vi "Destroy_MemBank.vi"(8 "error in":errorcluster, 11 "NNPC_MemBank_and_Params":T1={"MemBank_Data"={"MemBank"=variant, "MemBank Norm"=variant}, "PreProc_Options"={"DS_Name"="", "Input_Dims"={"C"=-1, "H"=-1, "W"=-1}, "Cropping"={"Left"=0.0, "Top"=0.0, "Right"=1.0, "Bottom"=1.0}, "Interpolation Type"=1, "MultiStage_ReSample?"=FALSE, "Dataset_Stats"={"means"={"R"=0.5385, "G"=0.5348, "B"=0.551}, "stds"={"R"=0.3673, "G"=0.3673, "B"=0.3505}}}, "Evaluation_Results"={"Threshold(Image)"=0.0, "Threshold(Pixel)"=0.0, "Pixel_Range"={"Min"=0.0, "Max"=0.0}}, "MemBank on GPU?"=FALSE} {"PreProc_Options"."Dataset_Stats"."stds"."R" format="%#_3g"; "PreProc_Options"."Dataset_Stats"."stds"."G" format="%#_3g"; "PreProc_Options"."Dataset_Stats"."stds"."B" format="%#_3g"; "PreProc_Options"."Dataset_Stats"."means"."R" format="%#_3g"; "PreProc_Options"."Dataset_Stats"."means"."G" format="%#_3g"; "PreProc_Options"."Dataset_Stats"."means"."B" format="%#_3g"; "PreProc_Options"."Interpolation Type" items=["Zero Order", "Bi-Linear", "Quadratic", "Cubic Spline"]; "Evaluation_Results"."Pixel_Range"."Min" format="%#_5g"}) -> (0 "error out":errorcluster)   [LabVIEW 2020]
uses:
  <vilib>/Ngene/DeepLTK Anomaly Detection Addon/Toolkit/API/Controls/MemBank_and_Norm_Variants.ctl
  <vilib>/Ngene/CuLab - GPU Accelerated Toolkit/Toolkit/Low_Level/Tensor_Classes/T_Children/T1D/T1D_Children/T1D_SGL/T1D_SGL.lvclass
  C:/Program Files/National Instruments/LabVIEW 2020/vi.lib/Ngene/CuLab - GPU Accelerated Toolkit/Toolkit/Low_Level/Tensor_Classes/Tensor.lvclass
  <vilib>/Ngene/CuLab - GPU Accelerated Toolkit/Toolkit/Low_Level/Tensor_Classes/T_Children/T2D/T2D_Children/T2D_SGL/T2D_SGL.lvclass
  <vilib>/Ngene/Deep Learning Toolkit/Toolkit/Deep_Learning_Toolkit_by_Ngene.lvlib
  <vilib>/Ngene/CuLab - GPU Accelerated Toolkit/Toolkit/CuLab.lvlib
  <vilib>/Ngene/DeepLTK Anomaly Detection Addon/Toolkit/DeepLTK_Anomaly_Detection_Addon.lvlib
  <vilib>/Ngene/DeepLTK Anomaly Detection Addon/Toolkit/API/Controls/NNPC_Evaluation_Results.ctl
  <vilib>/Ngene/Deep Learning Toolkit/Toolkit/NN_Data/API/NN_Dims(C,H,W).ctl
  <vilib>/Ngene/DeepLTK Anomaly Detection Addon/Toolkit/API/Controls/Image_Stats_RGB.ctl
  <vilib>/Ngene/DeepLTK Anomaly Detection Addon/Toolkit/API/Controls/NNPC_DS_Stats.ctl
  <vilib>/Ngene/DeepLTK Anomaly Detection Addon/Toolkit/API/Controls/Crop_CFG.ctl
  <vilib>/Ngene/DeepLTK Anomaly Detection Addon/Toolkit/API/Controls/NNPC_PreProcessing_Options.ctl
  Controls/NNPC_MemBank_and_Params.ctl
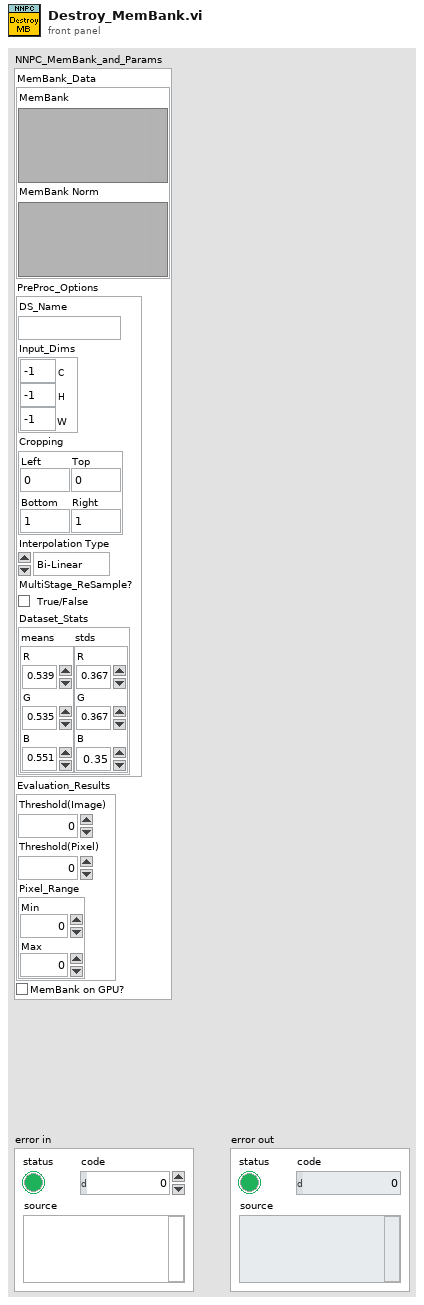
[diagram p1: front panel]
types:
  T1 = typedef "NNPC_MemBank_and_Params.ctl" = cluster{"MemBank_Data":T2, "PreProc_Options":T3, "Evaluation_Results":T8, "MemBank on GPU?":bool}
  T2 = typedef "DeepLTK_Anomaly_Detection_Addon.lvlib/MemBank_and_Norm_Variants.ctl" = cluster{"MemBank":variant, "MemBank Norm":variant}
  T3 = typedef "DeepLTK_Anomaly_Detection_Addon.lvlib/NNPC_PreProcessing_Options.ctl" = cluster{"DS_Name":string, "Input_Dims":T4, "Cropping":T5, "Interpolation Type":u32, "MultiStage_ReSample?":bool, "Dataset_Stats":T6}
  T4 = typedef "Deep_Learning_Toolkit_by_Ngene.lvlib/NN_Dims(C,H,W).ctl" = cluster{"C":i32, "H":i32, "W":i32}
  T5 = typedef "DeepLTK_Anomaly_Detection_Addon.lvlib/Crop_CFG.ctl" = cluster{"Left":sgl, "Top":sgl, "Right":sgl, "Bottom":sgl}
  T6 = typedef "DeepLTK_Anomaly_Detection_Addon.lvlib/NNPC_DS_Stats.ctl" = cluster{"means":T7, "stds":T7}
  T7 = typedef "DeepLTK_Anomaly_Detection_Addon.lvlib/Image_Stats_RGB.ctl" = cluster{"R":sgl, "G":sgl, "B":sgl}
  T8 = typedef "DeepLTK_Anomaly_Detection_Addon.lvlib/NNPC_Evaluation_Results.ctl" = cluster{"Threshold(Image)":sgl, "Threshold(Pixel)":sgl, "Pixel_Range":cluster{"Min":sgl, "Max":sgl}}
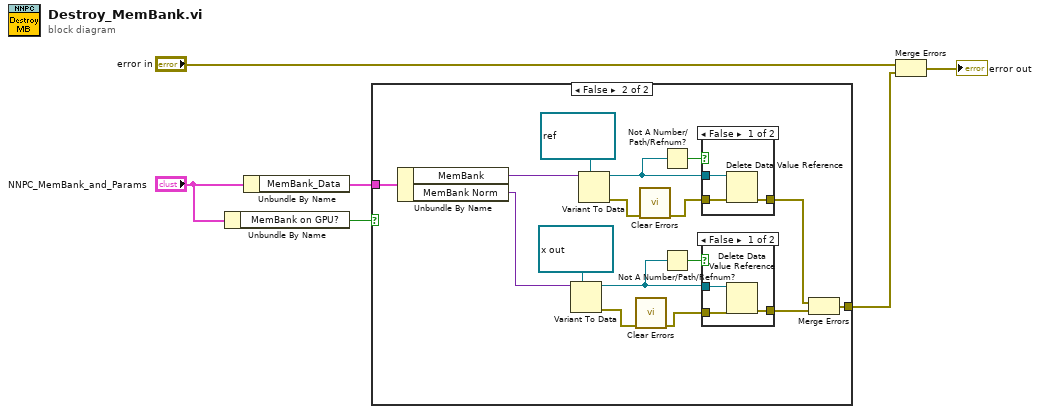
[diagram p0: block diagram]
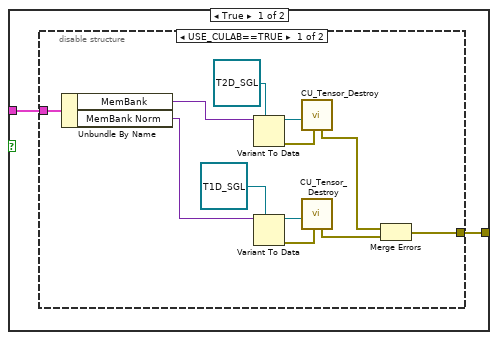
[diagram p2: hidden frame]
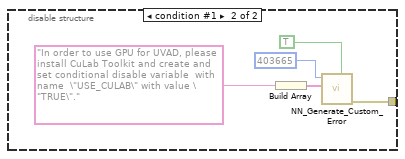
[diagram p3: hidden frame]
diagram:
  n1 = Unbundle By Name("NNPC_MemBank_and_Params") -> ("MemBank on GPU?"=w2:bool)
  n2 = Unbundle By Name("NNPC_MemBank_and_Params") -> ("MemBank_Data"=w1:T2)
  n3 = case shown="True" w2 {
    tunnel: w1 -> [w7 w27]
    tunnel: [w8 w26] -> w5
    frame True {
      n4 = disable-structure shown="USE_CULAB==TRUE" {
        disable-tunnel: [w11 w21] -> w8
        disable-tunnel: w7 -> [w20 _]
        frame condition #0 (active) {
          n5 = Unbundle By Name(w20) -> ("MemBank"=w18:variant, "MemBank Norm"=w16:variant)
          n6 = Variant To Data(type=refnum<class "T2D_SGL.lvclass"> refnum ("MemBank DVR"), Variant=w18) -> (data=w15:refnum<class "T2D_SGL.lvclass">, error out=w10:errorcluster)  [unwired: 1 in]
          n7 = Variant To Data(type=refnum<class "T1D_SGL.lvclass"> refnum ("Tensor in"), Variant=w16) -> (data=w14:refnum<class "T1D_SGL.lvclass">, error out=w9:errorcluster)  [unwired: 1 in]
          n8 = call <vilib>:"CU_Tensor_Destroy.vi"("error in (no error)"=w10, "Tensor in"=w15) -> ("error out"=w13:errorcluster)  [unwired: 9 in]
          n9 = call <vilib>:"CU_Tensor_Destroy.vi"("error in (no error)"=w9, "Tensor in"=w14) -> ("error out"=w12:errorcluster)  [unwired: 9 in]
          n10 = Merge Errors(w13, w12) -> (w11:errorcluster)
        }
        frame condition #1 {
          n11 = Build Array("In order to use GPU for UVAD, please install CuLab Toolkit and create and set conditional disable variable  with name  \"USE_CULAB\" with value \"TRUE\"." ("Message")) -> (w25:string[])
          n12 = call <vilib>:"NN_Generate_Custom_Error.vi"("show call chain? (TRUE)"=TRUE ("show call chain? (False)"), "Message"=w25, "Error_code"=403665) -> ("error out"=w21:errorcluster)  [unwired: 8 in]
        }
      }
    }
    frame False {
      n13 = Unbundle By Name(w27) -> ("MemBank"=w39:variant, "MemBank Norm"=w30:variant)
      n14 = Variant To Data(type=refnum<data-value> refnum ("MemBank Norm DVR"), Variant=w30) -> (data=w33:refnum<data-value>, error out=w31:errorcluster)  [unwired: 1 in]
      n15 = Variant To Data(type=refnum<data-value> refnum ("MemBank DVR"), Variant=w39) -> (data=w35:refnum<data-value>, error out=w32:errorcluster)  [unwired: 1 in]
      n16 = call <vilib>:"Clear Errors.vi"("error in (no error)"=w31) -> ("error out"=w29:errorcluster)  [unwired: 5 in, 1 out]
      n17 = call <vilib>:"Clear Errors.vi"("error in (no error)"=w32) -> ("error out"=w28:errorcluster)  [unwired: 5 in, 1 out]
      n18 = Not A Number/Path/Refnum?(number/path/refnum=w35) -> (NaN/Path/Refnum?=w40:bool)
      n19 = Not A Number/Path/Refnum?(number/path/refnum=w33) -> (NaN/Path/Refnum?=w41:bool)
      n20 = case shown="False" w40 {
        tunnel: [w44 w45] -> w37
        tunnel: w35 -> [w43 _]
        tunnel: w28 -> [w42 w45]
        frame False {
          n21 = Delete Data Value Reference(data value reference=w43, error in=w42) -> (error out=w44:errorcluster)  [unwired: 1 out]
        }
        frame True {
        }
      }
      n22 = case shown="False" w41 {
        tunnel: [w48 w49] -> w38
        tunnel: w33 -> [w47 _]
        tunnel: w29 -> [w46 w49]
        frame False {
          n23 = Delete Data Value Reference(data value reference=w47, error in=w46) -> (error out=w48:errorcluster)  [unwired: 1 out]
        }
        frame True {
        }
      }
      n24 = Merge Errors(w37, w38) -> (w26:errorcluster)
    }
  }
  n25 = Merge Errors("error in", w5) -> (→"error out":errorcluster)
